vi "Test Actor Messaging.vi"() -> ()   [LabVIEW 2026]
doc: "Run once. Sends Add 1, Add 5, Add -2, Reset, Add 3, then a normal stop. Expected Count 3, Processed 5, Stopped cleanly TRUE and no error."
uses:
  CounterActor/CounterActor.lvclass
  <vilib>/ActorFramework/Actor/Actor.lvclass
  Messages/Add/Counter Add Msg.lvclass
  Messages/Reset/Counter Reset Msg.lvclass
  <vilib>/ActorFramework/Stop Msg/Stop Msg.lvclass
panel:
  out "Messaging test passed":bool
  out "error out":errorcluster
  out "Stopped cleanly":bool
  out "Processed":dbl
  out "Count":dbl
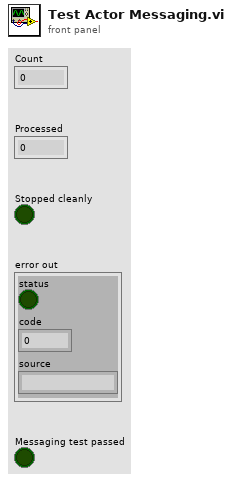
[diagram p1: front panel]
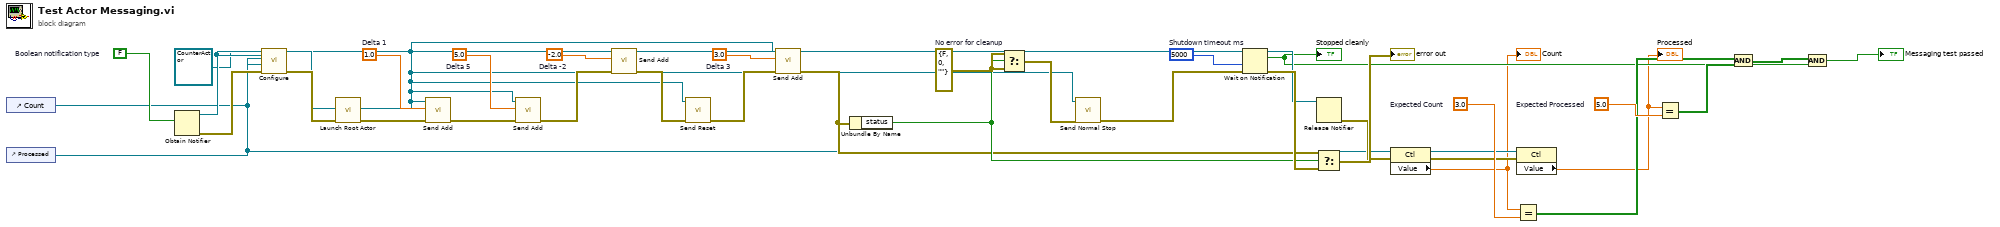
[diagram p0: block diagram]
diagram:
  w36 = 5.0  # Expected Processed
  w34 = 3.0  # Expected Count
  w27 = 5000  # Shutdown timeout ms
  w26 = errorcluster {"status"=FALSE, "code"=0, "source"=""}  # No error for cleanup
  w21 = 3.0  # Delta 3
  w18 = -2.0  # Delta -2
  w16 = 5.0  # Delta 5
  w14 = 1.0  # Delta 1
  w7 = FALSE  # Boolean notification type
  n1 = control-ref of="Count"() -> (w5:refnum<vi>)
  n2 = control-ref of="Processed"() -> (w6:refnum<vi>)
  n3 = Obtain Notifier(notification data type=w7) -> (notifier out=w8:refnum<notifier>, error out=w9:errorcluster)  [unwired: 3 in, 1 out]
  n4 = call "Configure.vi"("Stopped Notification"=w8, "error in"=w9, "Processed Display"=w6, "Count Display"=w5, "Actor in"=refnum<class "CounterActor.lvclass"> refnum ("CounterActor")) -> ("error out"=w11:errorcluster, "Actor out"=w10:refnum<class "CounterActor.lvclass">)  [unwired: 5 in]
  n5 = call <vilib>:"Launch Root Actor.vi"("error in (no error)"=w11, "Actor"=w10) -> ("error out"=w13:errorcluster, "Actor's Enqueuer"=w12:refnum<class "Message Enqueuer.lvclass">)  [unwired: 8 in]
  n6 = call "Send Add.vi"("error in (no error)"=w13, "Delta"=w14, "Message Enqueuer"=w12) -> ("error out"=w15:errorcluster)  [unwired: 7 in, 1 out]
  n7 = call "Send Add.vi"("error in (no error)"=w15, "Delta"=w16, "Message Enqueuer"=w12) -> ("error out"=w17:errorcluster)  [unwired: 7 in, 1 out]
  n8 = call "Send Add.vi"("error in (no error)"=w17, "Delta"=w18, "Message Enqueuer"=w12) -> ("error out"=w19:errorcluster)  [unwired: 7 in, 1 out]
  n9 = call "Send Reset.vi"("error in (no error)"=w19, "Message Enqueuer"=w12) -> ("error out"=w20:errorcluster)  [unwired: 8 in, 1 out]
  n10 = call "Send Add.vi"("error in (no error)"=w20, "Delta"=w21, "Message Enqueuer"=w12) -> ("error out"=w22:errorcluster)  [unwired: 7 in, 1 out]
  n11 = Unbundle By Name(w22) -> ("status"=w25:bool)
  n12 = Select(t=w26, s=w25, f=w26) -> (s? t:f=w24:errorcluster)
  n13 = call <vilib>:"Send Normal Stop.vi"("error in (no error)"=w24, "Message Enqueuer"=w12) -> ("error out"=w23:errorcluster)  [unwired: 9 in]
  n14 = Wait on Notification(notifier=w8, timeout in ms (-1)=w27, error in (no error)=w23) -> (notifier out=w28:refnum<notifier>, notification=w4:bool, error out=w29:errorcluster)  [unwired: 1 in, 1 out]
  "Stopped cleanly" <- w4
  n15 = Release Notifier(notifier=w28) -> (error out=w30:errorcluster)  [unwired: 2 in, 2 out]
  n16 = Select(t=w22, s=w25, f=w29) -> (s? t:f=→"error out":errorcluster)
  n17 = property class="Ctl"(reference=w5, error in=w30) -> (error out=w31:errorcluster, "Value"=w2:dbl)  [unwired: 1 out]
  "Count" <- w2
  n18 = property class="Ctl"(reference=w6, error in=w31) -> ("Value"=w3:dbl)  [unwired: 2 out]
  "Processed" <- w3
  n19 = Equal?(x=w2, y=w34) -> (x = y?=w33:bool[])
  n20 = Equal?(x=w3, y=w36) -> (x = y?=w35:bool[])
  n21 = And(x=w33, y=w35) -> (x .and. y?=w37:bool[])
  n22 = And(x=w37, y=w4) -> (x .and. y?=→"Messaging test passed":bool)
